vi "LinearFilter_ResetToValue.vi"(9 "InputValue":dbl, 11 "In LINEAR_FILTER":T1 {"Outputs" format="%13.5g"; "Inputs" format="%13.5g"; "OutputGains" format="%13.5g"; "InputGains" format="%13.5g"}) -> (3 "Out LINEAR_FILTER":T1 {"Outputs" format="%13.5g"; "Inputs" format="%13.5g"; "OutputGains" format="%13.5g"; "InputGains" format="%13.5g"})   [LabVIEW 2019, in "Trajectory_Library.lvlib"]
doc: "Reset the filter state. Sets the saved inputs and outputs to \"InputValue:\"\n\n\nInputs: \n - inLinearfilter - Linear filter data structure\n - InputValue - This value is used to fill the saved input and output values\n\nOutputs:\n - outLinearfilter - Updated linear filter data structurea"
uses:
  Trajectory_Library.lvlib
  TypeDef/LINEAR_FILTER.ctl
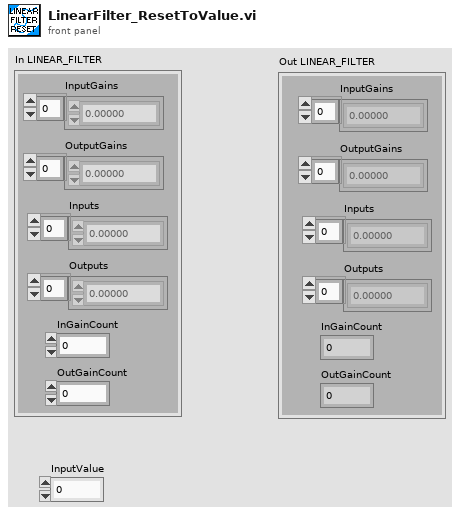
[diagram p1: front panel]
types:
  T1 = typedef "Trajectory_Library.lvlib/LINEAR_FILTER.ctl" = cluster{"InputGains":dbl[], "OutputGains":dbl[], "Inputs":dbl[], "Outputs":dbl[], "InGainCount":i32, "OutGainCount":i32}
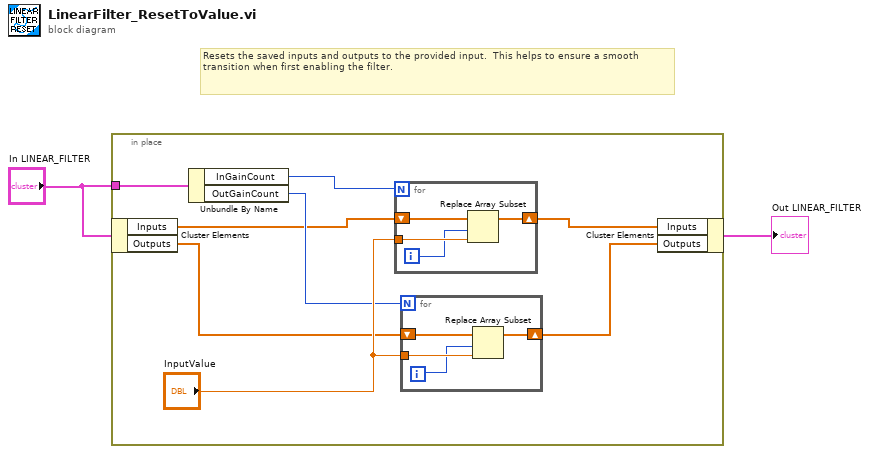
[diagram p0: block diagram]
diagram:
  # "Resets the saved inputs and outputs to the provided input.  This helps to ensure a smooth\ntransition when first enabling the filter."
  n1 = in-place {
    in-place-border: "In LINEAR_FILTER" -> [w7]
    n2 = in-place-cluster #1("In LINEAR_FILTER") -> ("Inputs"=w6:dbl[], "Outputs"=w5:dbl[])
    n3 = Unbundle By Name(w7) -> ("InGainCount"=w8:i32, "OutGainCount"=w9:i32)
    n4 = for {
      N: w8 -> [_]
      shift-right: [w17] -> w4
      shift-left: w6 -> [w18]
      tunnel: "InputValue" -> [w16]
      i -> [w15]
      n5 = Replace Array Subset(array=w18, new element=w16, index=w15) -> (w17:dbl[])
    }
    n6 = for {
      N: w9 -> [_]
      shift-right: [w13] -> w3
      shift-left: w5 -> [w14]
      tunnel: "InputValue" -> [w12]
      i -> [w11]
      n7 = Replace Array Subset(array=w14, new element=w12, index=w11) -> (w13:dbl[])
    }
    n8 = in-place-cluster #1("Inputs"=w4, "Outputs"=w3) -> (→"Out LINEAR_FILTER":T1)
  }
